vi "RDV-handle-AnalyseAllPermittivityError.vi"(7 "%?":bool, 10 "Compare Array":cluster{"ref":i32, "Set":i32}[](array[cluster])=[{"ref"=0, "Set"=0}, {"ref"=3, "Set"=1}, {"ref"=3, "Set"=2}], 11 "RDV-Reflection_Data_viewer in":refnum<class "RDV-Reflection_Data_viewer.lvclass">) -> (0 "Total Error Imag":dbl[](array[numeric]), 1 "Total Error real":dbl[](array[numeric]), 2 "All Error imag":dbl[][](array[numeric]), 3 "All Error real":dbl[][](array[numeric]), 4 "Total Error":dbl[](array[numeric]))   [LabVIEW 2020, in "RDV-Reflection_Data_viewer.lvclass"]
doc: "Runs RDV-handle-AnalysePermittivityError for every entry of Compare Array. Returns the real, imaginary and total errors per entry and in all."
uses:
  RDV-Reflection_Data_viewer.lvclass
  RDV-Reflection_Data_viewer.lvclass/RDV-Reflection_Data_viewer.ctl
  7787610a-5379-4eb4-852a-f3ed590529b8.vi
  ed438d76-670c-41f2-8cec-239e2b830610.vi
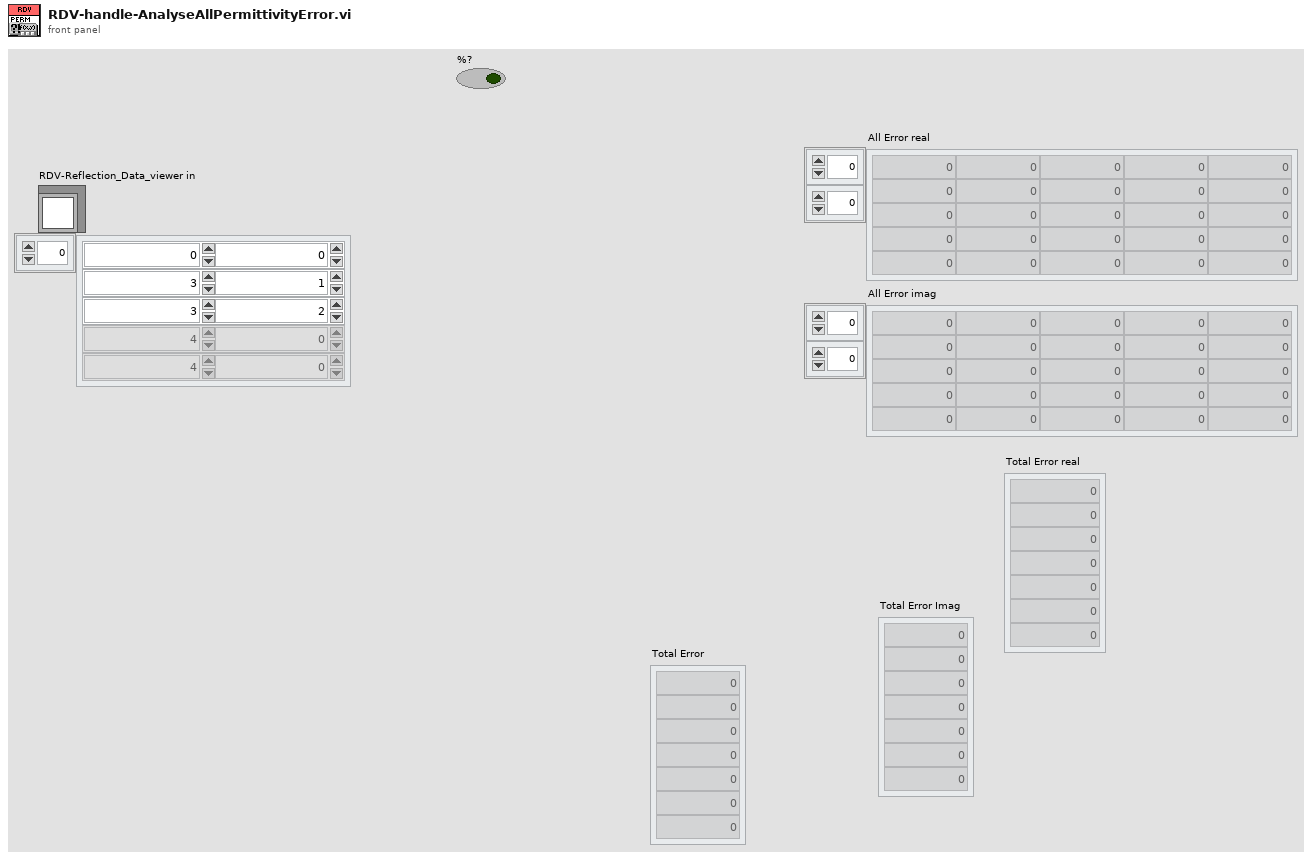
[diagram p1: front panel]
types:
  T1 = typedef "RDV-Reflection_Data_viewer.lvclass/RDV-UPDATE_IGNORE_LIST.ctl" = string[]
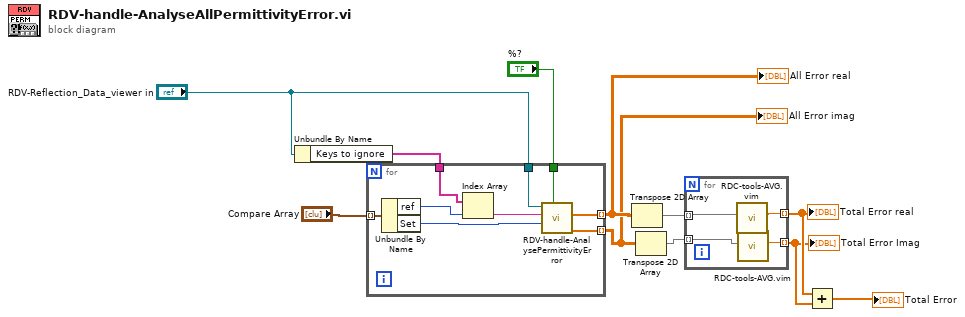
[diagram p0: block diagram]
diagram:
  n1 = Unbundle By Name("RDV-Reflection_Data_viewer in") -> ("Keys to ignore"=w9:T1)
  n2 = for {
    tunnel: "RDV-Reflection_Data_viewer in" -> [w20]
    tunnel: "Compare Array" -> [w19] mode=indexing
    tunnel: w9 -> [w17]
    tunnel: [w14] -> w2 mode=indexing
    tunnel: [w13] -> w1 mode=indexing
    tunnel: "%?" -> [w12]
    n3 = Unbundle By Name(w19) -> ("ref"=w18:i32, "Set"=w15:i32)
    n4 = Index Array(array=w17, index=w18) -> (element=w16:string)
    n5 = call "RDV-handle-AnalysePermittivityError.vi"("%?"=w12, "set"=w15, "Reference key"=w16, "RDV-Reflection_Data_viewer in"=w20) -> ("imag Error"=w13:dbl[], "real error"=w14:dbl[])  [unwired: 4 in, 2 out]
  }
  "All Error imag" <- w1
  "All Error real" <- w2
  n6 = Transpose 2D Array(2D array=w2) -> (transposed array=w8:dbl[][])
  n7 = Transpose 2D Array(2D array=w1) -> (transposed array=w7:dbl[][])
  n8 = for {
    tunnel: w8 -> [w24] mode=indexing
    tunnel: [w23] -> w6 mode=indexing
    tunnel: w7 -> [w22] mode=indexing
    tunnel: [w21] -> w5 mode=indexing
    n9 = call "RDC-tools-AVG.vim"("Data Array"=w24) -> ("AVG"=w23:dbl)  [unwired: 10 in]
    n10 = call "RDC-tools-AVG.vim"("Data Array"=w22) -> ("AVG"=w21:dbl)  [unwired: 10 in]
  }
  "Total Error real" <- w6
  "Total Error Imag" <- w5
  n11 = Add(x=w6, y=w5) -> (x+y=→"Total Error":dbl[])
